vi "GIT-Current Local Branches.vi"(8 "error in":errorcluster, 11 "Path":path) -> (0 "error out":errorcluster, 2 "branches":string[](array[string]))   [LabVIEW 2017]
doc: "show the current branch name\n\nNote: Set the \"Working Dir\" through the Git-API accessor (property node) to tell git where - in which directory - to execute this command.\n\n____\nHAMPEL SOFTWARE ENGINEERING v2.0.2 (2022-02-01 15:19)"
panel:
  out "std out":string
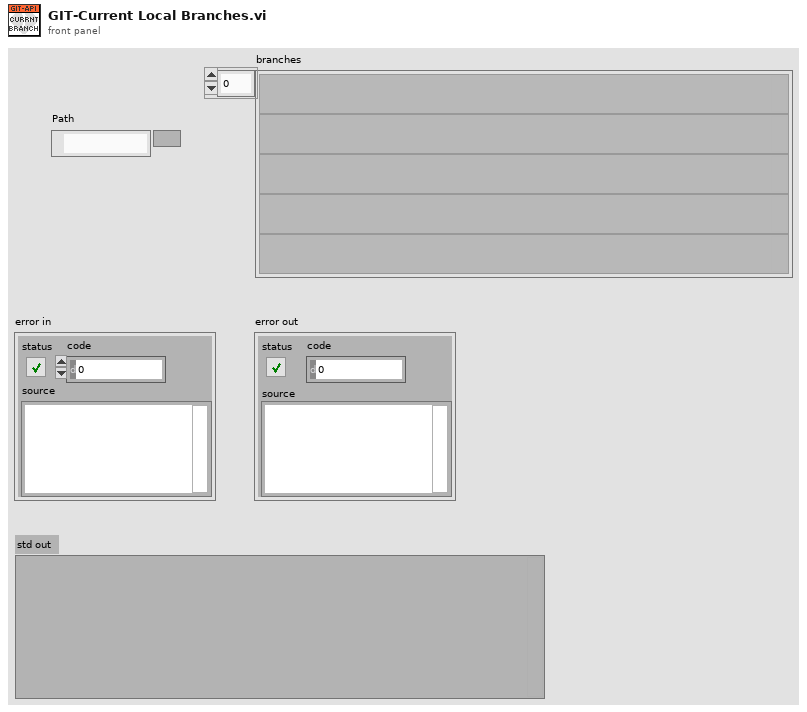
[diagram p1: front panel]
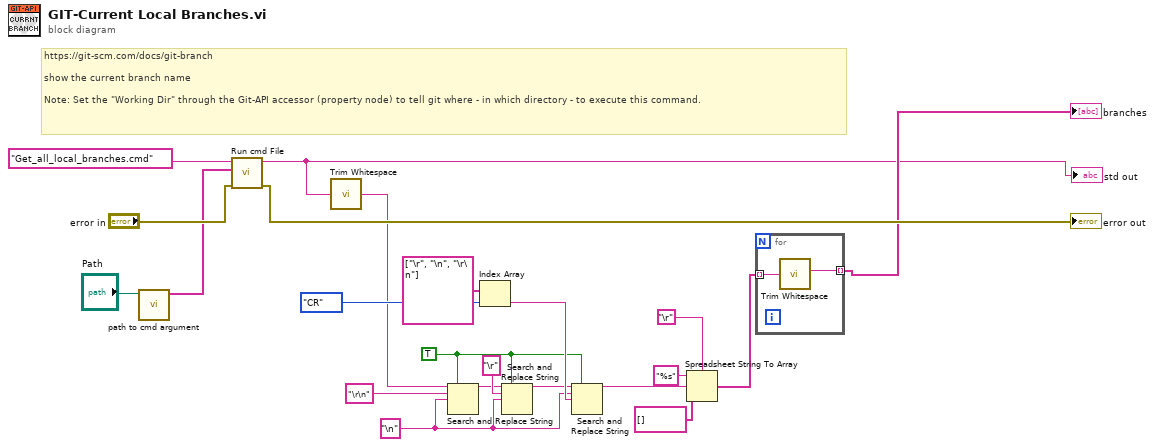
[diagram p0: block diagram]
diagram:
  w14 = TRUE ("replace all? (F)")
  w16 = "\n" ("search string")
  # "https://git-scm.com/docs/git-branch\n\nshow the current branch name\n\nNote: Set the \"Working Dir\" through the Git-API accessor (property node) to tell git where - in which directory - to execute this command."
  n1 = call "path to cmd argument.vi"("path"="Path") -> ("Array"=w1:string[])  [unwired: 10 in]
  n2 = call "Run cmd File.vi"("Error in"="error in", "args"=w1, "name or relative path"="Get_all_local_branches.cmd") -> ("Error out"=→"error out":errorcluster, "standard output"=w4:string)  [unwired: 6 in, 1 out]
  "std out" <- w4
  n3 = call <vilib>:"Trim Whitespace.vi"("string"=w4) -> ("trimmed string"=w3:string)  [unwired: 1 in]
  n4 = Search and Replace String(replace all?=w14, input string=w3, search string="\r\n", replace string=w16) -> (result string=w11:string)  [unwired: 4 in, 3 out]
  n5 = Index Array(array=string[] ["\r", "\n", "\r\n"], index=enum16{"CR", "LF", "CRLF"}."CR" ("Convert to:")) -> (element=w18:string)
  n6 = Search and Replace String(replace all?=w14, input string=w11, search string="\r", replace string=w16) -> (result string=w13:string)  [unwired: 4 in, 3 out]
  n7 = Search and Replace String(replace all?=w14, input string=w13, search string=w16, replace string=w18) -> (result string=w21:string)  [unwired: 4 in, 3 out]
  n8 = Spreadsheet String To Array(delimiter (Tab)="\r" ("Carriage Return Constant"), format string="%s", spreadsheet string=w21, array type (2D Dbl)=string[] [] ("Array of Strings")) -> (array=w20:string[])
  n9 = for {
    tunnel: [w24] -> w5 mode=indexing
    tunnel: w20 -> [w23] mode=indexing
    n10 = call <vilib>:"Trim Whitespace.vi"("string"=w23) -> ("trimmed string"=w24:string)  [unwired: 1 in]
  }
  "branches" <- w5
